vi "ReversedEngineering CreateEdges.vi"(1 "NodeRef":refnum<class "AbstractNode.lvclass">, 2 "AllNodes":refnum<class "AbstractNode.lvclass">[](array[class]), 3 "NodeClassInfo":T1, 5 "error in (no error)":errorcluster, 6 "Show Multiplicity":bool=TRUE) -> (15 "EdgesCreated":refnum<class "AbstractEdge.lvclass">[](array[class]), 19 "error out":errorcluster)   [LabVIEW 2020]
uses:
  <resource>/Framework/Providers/Open_GDS/UML/AbstractEdge_class/AbstractEdge.lvclass
  <resource>/Framework/Providers/Open_GDS/UML/AbstractNode_class/AbstractNode.lvclass
  <resource>/Framework/Providers/Open_GDS/UML/ReversedEngineering/ReversedEngineering ClassInfoType.ctl
  <resource>/Framework/Providers/Open_GDS/ClassProviders/Common/CommonVIs/CommonVIs_VisibilityType.ctl
  <resource>/Framework/Providers/Open_GDS/ClassProviders/Common/CommonVIs/CommonVIs_AttributeInfoType.ctl
  <resource>/Framework/Providers/Open_GDS/ClassProviders/Common/CommonVIs/CommonVIs_AttributeDataType.ctl
  <resource>/Framework/Providers/Open_GDS/UML/ReversedEngineering/ReversedEngineering_ClassDependencyDetailsType.ctl
  <resource>/Framework/Providers/Open_GDS/ClassProviders/Common/ScriptingFunctions/SubVIs/Scripting_ViDependencyType.ctl
  <resource>/Framework/Providers/Open_GDS/UML/ClassRelationshipEdge_class/ClassRelationshipEdge.lvclass
  C:/Program Files (x86)/National Instruments/LabVIEW 2020/resource/Framework/Providers/Open_GDS/UML/AbstractEdge_class/AbstractEdge.lvclass
  <resource>/Framework/Providers/Open_GDS/UML/ClassRelationshipEdge_class/ExternaSetParamType.ctl
  <resource>/Framework/Providers/Open_GDS/UML/ArrowHead_class/ArrowHeadType.ctl
  <resource>/Framework/Providers/Open_GDS/UML/BentStyle_class/BentStyleType.ctl
  <resource>/Framework/Providers/Open_GDS/UML/LineStyle_class/LineStyleType.ctl
  <resource>/Framework/Providers/Open_GDS/UML/ReversedEngineering/ReversedEngineering_ViDependencyDetailsType.ctl
  <resource>/Framework/Providers/Open_GDS/UML/ArrowHead_class/ArrowHead.lvclass
  <resource>/Framework/Providers/Open_GDS/UML/BentStyle_class/BentStyle.lvclass
  <resource>/Framework/Providers/Open_GDS/UML/LineStyle_class/LineStyle.lvclass
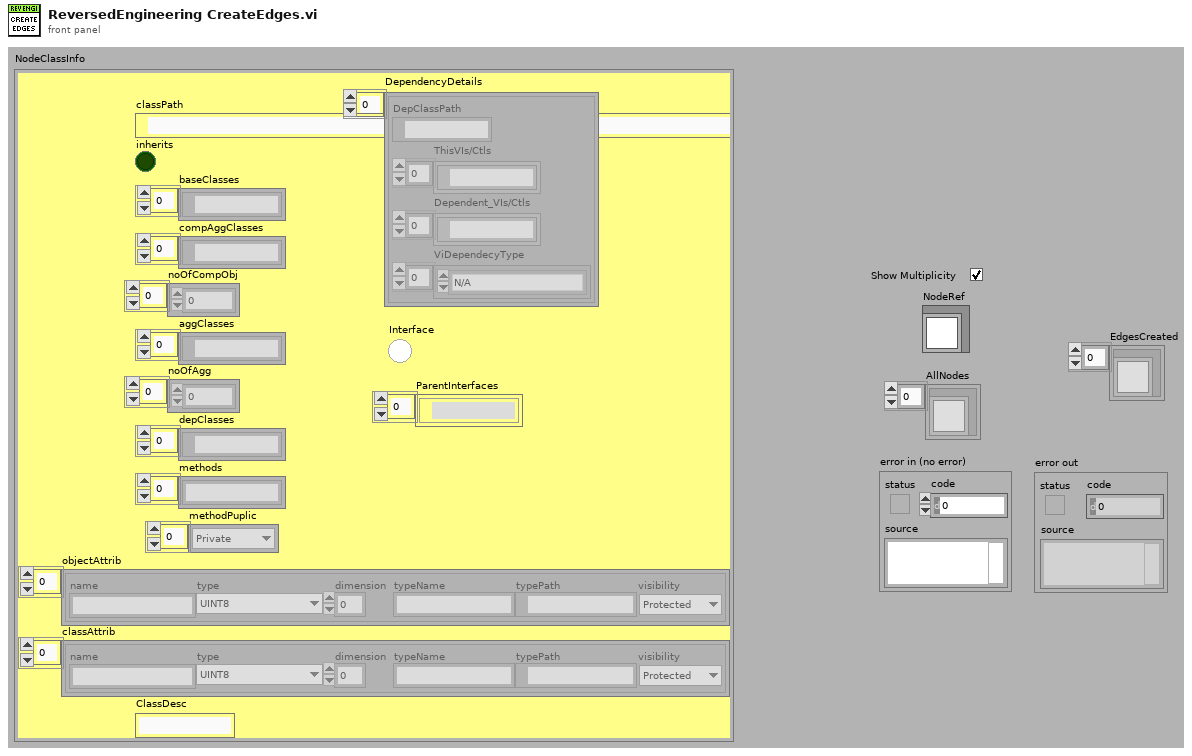
[diagram p1: front panel]
types:
  T1 = typedef "ReversedEngineering ClassInfoType.ctl" = cluster{"classPath":path, "inherits":bool, "baseClasses":path[], "compAggClasses":path[], "noOfCompObj":i32[], "aggClasses":path[], "noOfAgg":i32[], "depClasses":path[], "methods":string[], "methodPuplic":T2[], "objectAttrib":T3[], "classAttrib":T3[], "ClassDesc":string, "DependencyDetails":T5[], "Interface":bool, "ParentInterfaces":path[]}
  T2 = typedef "CommonVIs_VisibilityType.ctl" = enum16{"Public", "Private", "Protected"}
  T3 = typedef "CommonVIs_AttributeInfoType.ctl" = cluster{"name":string, "type":T4, "dimension":i32, "typeName":string, "typePath":path, "visibility":T2}
  T4 = typedef "CommonVIs_AttributeDataType.ctl" = enum16{"UINT8", "INT8", "UINT16", "INT16", "UINT32", "INT32", "UINT64", "INT64", "SGL", "DBL", "EXT", "CSG", "CDB", "CXT", "TimeStamp", "STRING", "PATH", "BOOL", "ENUM", "RefNum", "VIRefNum", "LabVIEW Class", "Cluster", "Variant", "TypeDef", "Waveform", "LabVIEW Object", "Other", "void", "Set", "Map"}
  T5 = typedef "ReversedEngineering_ClassDependencyDetailsType.ctl" = cluster{"DepClassPath":path, "ThisVIs/Ctls":path[], "Dependent_VIs/Ctls":path[], "ViDependecyType":T6[]}
  T6 = typedef "Scripting_ViDependencyType.ctl" = enum16{"N/A", "Launches"}
  T7 = typedef "ReversedEngineering_ViDependencyDetailsType.ctl" = cluster{"ThisVIs/Ctls":path[], "Dependent_VIs/Ctls":path[]}
  T8 = typedef "BentStyle.lvclass/BentStyleType.ctl" = enum16{"STRAIGHT", "HV", "VH", "HVH", "VHV", "ARC"}
  T9 = typedef "ClassRelationshipEdge.lvclass/ExternaSetParamType.ctl" = enum16{"StartLabel", "MidLabel", "EndLabel", "StartNode", "EndNode", "BendType", "StartArrow", "EndArrow", "StartOffset", "EndOffset", "LineStyle"}
  T10 = typedef "ArrowHead.lvclass/ArrowHeadType.ctl" = enum16{"NONE", "TRIANGLE", "BLACK_TRIANGLE", "V", "HALF_V", "DIAMOND", "BLACK_DIAMOND"}
  T11 = typedef "LineStyle.lvclass/LineStyleType.ctl" = enum16{"SOLID", "DOTTED"}
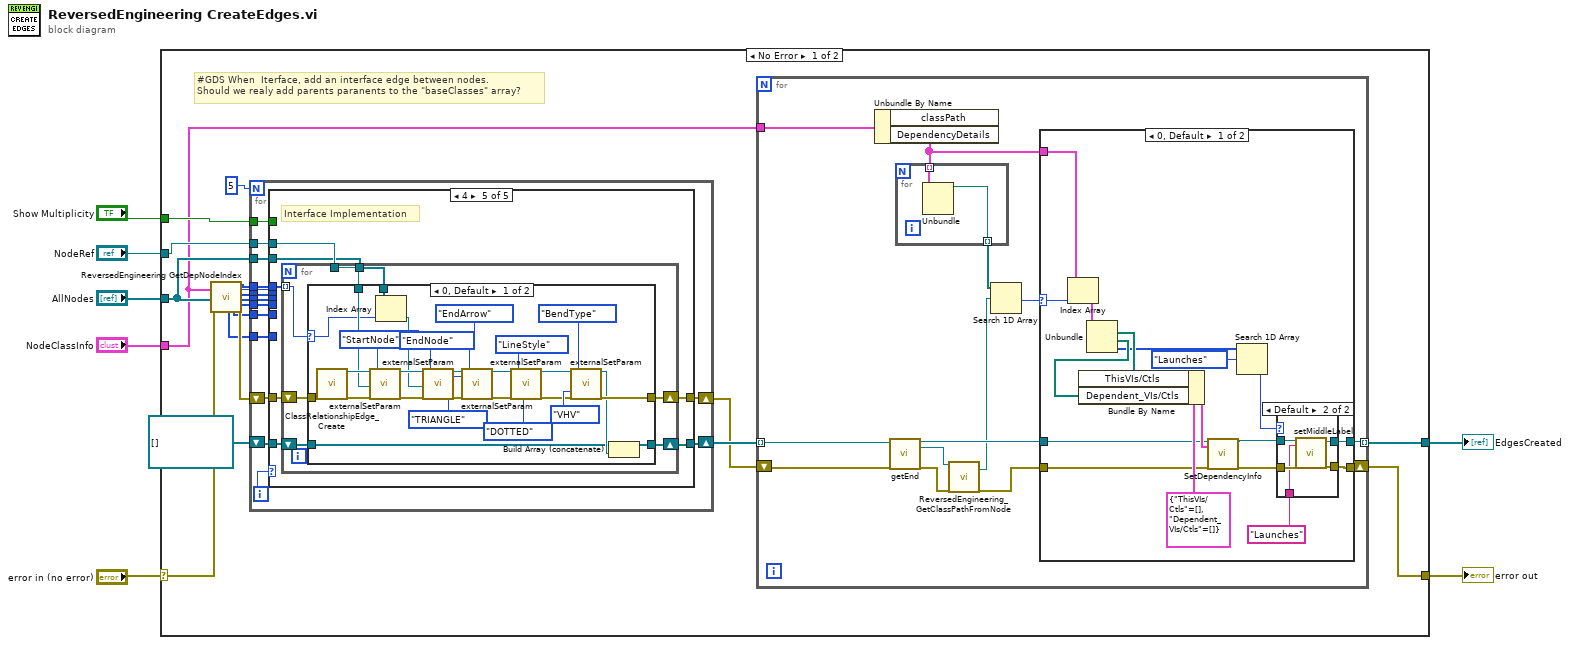
[diagram p0: block diagram]
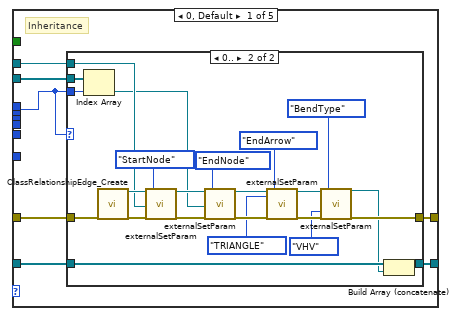
[diagram p4: hidden frame]
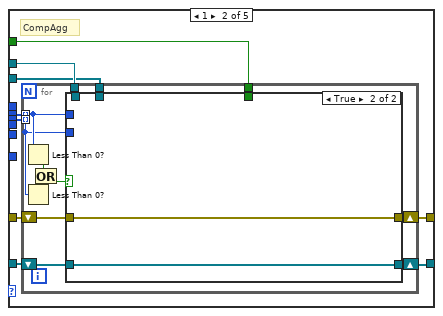
[diagram p6: hidden frame]
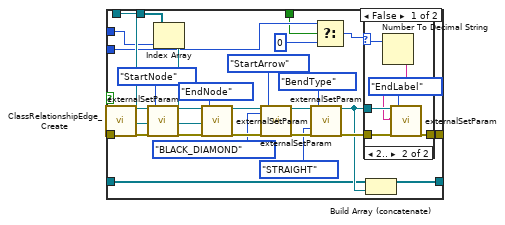
[diagram p7: hidden frame]
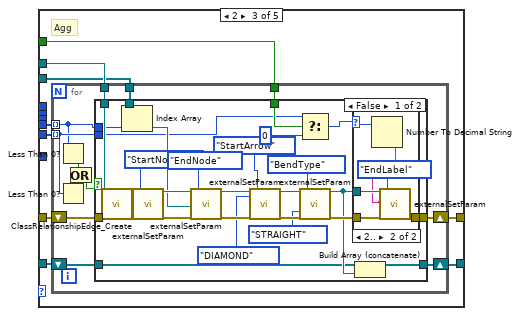
[diagram p9: hidden frame]
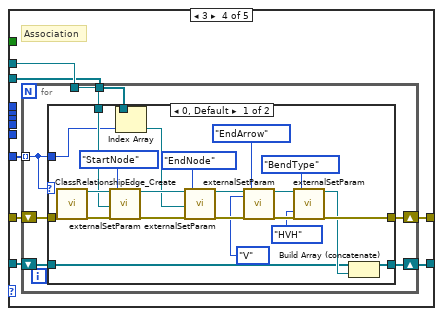
[diagram p12: hidden frame]
diagram:
  n1 = case shown="No Error" "error in (no error)" {
    selector: "error in (no error)" -> [w17 w313]
    tunnel: [w9 w313] -> w6
    tunnel: [w12 _] -> w5
    tunnel: "Show Multiplicity" -> [w16 _]
    tunnel: "AllNodes" -> [w14 _]
    tunnel: "NodeRef" -> [w15 _]
    tunnel: "NodeClassInfo" -> [w11 _]
    frame No Error {
      # "#GDS When  Iterface, add an interface edge between nodes.\nShould we realy add parents paranents to the \"baseClasses\" array?"
      n2 = call <resource>:"ReversedEngineering GetDepNodeIndex.vi"("classInfo"=w11, "AllNodes"=w14, "error in (no error)"=w17) -> ("depNodes"=w19:i32[], "noOfAgg"=w20:i32[], "InterfaceNodes"=w8:i32[], "inheritanceNode"=w24:i32, "compAggNodes"=w23:i32[], "noOfCompAgg"=w22:i32[], "aggNodes"=w21:i32[], "error out"=w25:errorcluster)  [unwired: 1 in, 8 out]
      n3 = for {
        N: 5 -> [_]
        tunnel: w15 -> [w82]
        shift-right: [w80] -> w10
        shift-left: w25 -> [w81]
        tunnel: w14 -> [w78]
        tunnel: w24 -> [w77]
        shift-right: [w76] -> w13
        shift-left: refnum<class "ClassRelationshipEdge.lvclass">[] [] ("empty") -> [w75]
        tunnel: w23 -> [w74]
        tunnel: w22 -> [w73]
        tunnel: w21 -> [w72]
        tunnel: w20 -> [w71]
        tunnel: w19 -> [w70]
        tunnel: w16 -> [w69]
        tunnel: w8 -> [w68]
        i -> [w79]
        n4 = case shown="4" w79 {
          tunnel: w81 -> [w89 w123 w181 w237 w276]
          tunnel: w82 -> [w88 w122 w180 w236 w275]
          tunnel: [w84 w121 w179 w235 w274] -> w80
          tunnel: w78 -> [w87 w119 w178 w234 w273]
          tunnel: w77 -> [w83 _ _ _ _]
          tunnel: [w86 w116 w176 w232 w271] -> w76
          tunnel: w75 -> [w85 w117 w177 w233 w272]
          tunnel: w74 -> [_ w120 _ _ _]
          tunnel: w73 -> [_ w118 _ _ _]
          tunnel: w72 -> [_ _ w175 _ _]
          tunnel: w71 -> [_ _ w174 _ _]
          tunnel: w70 -> [_ _ _ w231 _]
          tunnel: w69 -> [_ w115 w173 _ _]
          tunnel: w68 -> [_ _ _ _ w270]
          frame 0, Default {
            # "Inheritance"
            n5 = case shown="0.." w83 {
              tunnel: w89 -> [w91 w114]
              tunnel: w88 -> [_ w105]
              tunnel: w87 -> [_ w104]
              tunnel: w83 -> [_ w103]
              tunnel: [w90 w99] -> w86
              tunnel: w85 -> [w90 w98]
              tunnel: [w91 w95] -> w84
              frame Default {
              }
              frame 0.. {
                n6 = Index Array(array=w104, index=w103) -> (element=w102:refnum<class "AbstractNode.lvclass">)
                n7 = call <resource>:"ClassRelationshipEdge_Create.vi"("error in (no error)"=w114) -> ("reference out"=w113:refnum<class "ClassRelationshipEdge.lvclass">, "error out"=w112:errorcluster)  [unwired: 1 in, 16 out]
                n8 = call-dynamic "externalSetParam.vi"("reference"=w113, "node"=w105, "error in (no error)"=w112, "setParam"=ExternaSetParamType."StartNode") -> ("reference out"=w110:refnum<class "ClassRelationshipEdge.lvclass">, "error out"=w109:errorcluster)  [unwired: 14 in]
                n9 = call-dynamic "externalSetParam.vi"("reference"=w110, "node"=w102, "error in (no error)"=w109, "setParam"=ExternaSetParamType."EndNode") -> ("reference out"=w108:refnum<class "ClassRelationshipEdge.lvclass">, "error out"=w107:errorcluster)  [unwired: 14 in]
                n10 = call-dynamic "externalSetParam.vi"("reference"=w108, "arrowHead"=ArrowHeadType."TRIANGLE", "error in (no error)"=w107, "setParam"=ExternaSetParamType."EndArrow") -> ("reference out"=w97:refnum<class "ClassRelationshipEdge.lvclass">, "error out"=w96:errorcluster)  [unwired: 14 in]
                n11 = call-dynamic "externalSetParam.vi"("reference"=w97, "bentStyle"=BentStyleType."VHV", "error in (no error)"=w96, "setParam"=ExternaSetParamType."BendType") -> ("reference out"=w94:refnum<class "ClassRelationshipEdge.lvclass">, "error out"=w95:errorcluster)  [unwired: 14 in]
                n12 = Build Array (concatenate)(w98, w94) -> (w99:refnum<class "ClassRelationshipEdge.lvclass">[])
              }
            }
          }
          frame 1 {
            # "CompAgg"
            n13 = for {
              shift-right: [w133] -> w121
              shift-left: w123 -> [w135]
              tunnel: w122 -> [w134]
              tunnel: w120 -> [w128] mode=indexing
              tunnel: w119 -> [w132]
              tunnel: w118 -> [w127] mode=indexing
              shift-right: [w130] -> w116
              shift-left: w117 -> [w131]
              tunnel: w115 -> [w129]
              n14 = Less Than 0?(x=w128) -> (x < 0?=w126:bool)
              n15 = Less Than 0?(x=w127) -> (x < 0?=w125:bool)
              n16 = Or(x=w126, y=w125) -> (x .or. y?=w124:bool)
              n17 = case shown="True" w124 {
                tunnel: w135 -> [w152 w172]
                tunnel: w134 -> [w151 _]
                tunnel: [w150 w172] -> w133
                tunnel: w128 -> [w149 _]
                tunnel: w132 -> [w148 _]
                tunnel: w131 -> [w142 w171]
                tunnel: [w141 w171] -> w130
                tunnel: w127 -> [w138 _]
                tunnel: w129 -> [w137 _]
                frame False {
                  n18 = call <resource>:"ClassRelationshipEdge_Create.vi"("error in (no error)"=w152) -> ("reference out"=w163:refnum<class "ClassRelationshipEdge.lvclass">, "error out"=w162:errorcluster)  [unwired: 1 in, 16 out]
                  n19 = call-dynamic "externalSetParam.vi"("reference"=w163, "node"=w151, "error in (no error)"=w162, "setParam"=ExternaSetParamType."StartNode") -> ("reference out"=w160:refnum<class "ClassRelationshipEdge.lvclass">, "error out"=w159:errorcluster)  [unwired: 14 in]
                  n20 = Index Array(array=w148, index=w149) -> (element=w147:refnum<class "AbstractNode.lvclass">)
                  n21 = call-dynamic "externalSetParam.vi"("reference"=w160, "node"=w147, "error in (no error)"=w159, "setParam"=ExternaSetParamType."EndNode") -> ("reference out"=w158:refnum<class "ClassRelationshipEdge.lvclass">, "error out"=w157:errorcluster)  [unwired: 14 in]
                  n22 = call-dynamic "externalSetParam.vi"("reference"=w158, "arrowHead"=ArrowHeadType."BLACK_DIAMOND", "error in (no error)"=w157, "setParam"=ExternaSetParamType."StartArrow") -> ("reference out"=w156:refnum<class "ClassRelationshipEdge.lvclass">, "error out"=w155:errorcluster)  [unwired: 14 in]
                  n23 = call-dynamic "externalSetParam.vi"("reference"=w156, "bentStyle"=BentStyleType."STRAIGHT", "error in (no error)"=w155, "setParam"=ExternaSetParamType."BendType") -> ("reference out"=w143:refnum<class "ClassRelationshipEdge.lvclass">, "error out"=w154:errorcluster)  [unwired: 14 in]
                  n24 = Select(t=w138, s=w137, f=0) -> (s? t:f=w139:i32)
                  n25 = case shown="2.." w139 {
                    selector: w139 -> [_ w167]
                    tunnel: w143 -> [_ w170]
                    tunnel: w154 -> [w164 w169]
                    tunnel: [w164 w168] -> w150
                    frame 0, Default {
                    }
                    frame 2.. {
                      n26 = Number To Decimal String(number=w167) -> (decimal integer string=w166:string)  [unwired: 1 out]
                      n27 = call-dynamic "externalSetParam.vi"("reference"=w170, "string"=w166, "error in (no error)"=w169, "setParam"=ExternaSetParamType."EndLabel") -> ("error out"=w168:errorcluster)  [unwired: 14 in, 1 out]
                    }
                  }
                  n28 = Build Array (concatenate)(w142, w143) -> (w141:refnum<class "ClassRelationshipEdge.lvclass">[])
                }
                frame True {
                }
              }
            }
          }
          frame 2 {
            # "Agg"
            n29 = for {
              shift-right: [w191] -> w179
              shift-left: w181 -> [w193]
              tunnel: w180 -> [w192]
              tunnel: w175 -> [w183] mode=indexing
              tunnel: w178 -> [w190]
              tunnel: w174 -> [w184] mode=indexing
              shift-right: [w188] -> w176
              shift-left: w177 -> [w189]
              tunnel: w173 -> [w187]
              n30 = Less Than 0?(x=w183) -> (x < 0?=w186:bool)
              n31 = Less Than 0?(x=w184) -> (x < 0?=w185:bool)
              n32 = Or(x=w186, y=w185) -> (x .or. y?=w182:bool)
              n33 = case shown="False" w182 {
                tunnel: w193 -> [w210 w230]
                tunnel: w192 -> [w209 _]
                tunnel: [w208 w230] -> w191
                tunnel: w190 -> [w207 _]
                tunnel: w189 -> [w200 w229]
                tunnel: [w199 w229] -> w188
                tunnel: w187 -> [w196 _]
                tunnel: w184 -> [w195 _]
                tunnel: w183 -> [w194 _]
                frame False {
                  n34 = call <resource>:"ClassRelationshipEdge_Create.vi"("error in (no error)"=w210) -> ("reference out"=w221:refnum<class "ClassRelationshipEdge.lvclass">, "error out"=w220:errorcluster)  [unwired: 1 in, 16 out]
                  n35 = Index Array(array=w207, index=w194) -> (element=w206:refnum<class "AbstractNode.lvclass">)
                  n36 = call-dynamic "externalSetParam.vi"("reference"=w221, "node"=w209, "error in (no error)"=w220, "setParam"=ExternaSetParamType."StartNode") -> ("reference out"=w218:refnum<class "ClassRelationshipEdge.lvclass">, "error out"=w217:errorcluster)  [unwired: 14 in]
                  n37 = call-dynamic "externalSetParam.vi"("reference"=w218, "node"=w206, "error in (no error)"=w217, "setParam"=ExternaSetParamType."EndNode") -> ("reference out"=w216:refnum<class "ClassRelationshipEdge.lvclass">, "error out"=w215:errorcluster)  [unwired: 14 in]
                  n38 = call-dynamic "externalSetParam.vi"("reference"=w216, "arrowHead"=ArrowHeadType."DIAMOND", "error in (no error)"=w215, "setParam"=ExternaSetParamType."StartArrow") -> ("reference out"=w214:refnum<class "ClassRelationshipEdge.lvclass">, "error out"=w213:errorcluster)  [unwired: 14 in]
                  n39 = Select(t=w195, s=w196, f=0) -> (s? t:f=w197:i32)
                  n40 = call-dynamic "externalSetParam.vi"("reference"=w214, "bentStyle"=BentStyleType."STRAIGHT", "error in (no error)"=w213, "setParam"=ExternaSetParamType."BendType") -> ("reference out"=w201:refnum<class "ClassRelationshipEdge.lvclass">, "error out"=w212:errorcluster)  [unwired: 14 in]
                  n41 = case shown="2.." w197 {
                    selector: w197 -> [_ w225]
                    tunnel: w201 -> [_ w228]
                    tunnel: w212 -> [w222 w227]
                    tunnel: [w222 w226] -> w208
                    frame 0, Default {
                    }
                    frame 2.. {
                      n42 = Number To Decimal String(number=w225) -> (decimal integer string=w224:string)  [unwired: 1 out]
                      n43 = call-dynamic "externalSetParam.vi"("reference"=w228, "string"=w224, "error in (no error)"=w227, "setParam"=ExternaSetParamType."EndLabel") -> ("error out"=w226:errorcluster)  [unwired: 14 in, 1 out]
                    }
                  }
                  n44 = Build Array (concatenate)(w200, w201) -> (w199:refnum<class "ClassRelationshipEdge.lvclass">[])
                }
                frame True {
                }
              }
            }
          }
          frame 3 {
            # "Association"
            n45 = for {
              shift-right: [w242] -> w235
              shift-left: w237 -> [w244]
              tunnel: w236 -> [w243]
              tunnel: w234 -> [w241]
              shift-right: [w239] -> w232
              shift-left: w233 -> [w240]
              tunnel: w231 -> [w238] mode=indexing
              n46 = case shown="0, Default" w238 {
                tunnel: w244 -> [w257 w269]
                tunnel: w243 -> [w256 _]
                tunnel: [w255 w269] -> w242
                tunnel: w241 -> [w254 _]
                tunnel: w240 -> [w247 w268]
                tunnel: [w246 w268] -> w239
                tunnel: w238 -> [w245 _]
                frame 0, Default {
                  n47 = call <resource>:"ClassRelationshipEdge_Create.vi"("error in (no error)"=w257) -> ("reference out"=w267:refnum<class "ClassRelationshipEdge.lvclass">, "error out"=w266:errorcluster)  [unwired: 1 in, 16 out]
                  n48 = call-dynamic "externalSetParam.vi"("reference"=w267, "node"=w256, "error in (no error)"=w266, "setParam"=ExternaSetParamType."StartNode") -> ("reference out"=w264:refnum<class "ClassRelationshipEdge.lvclass">, "error out"=w263:errorcluster)  [unwired: 14 in]
                  n49 = Index Array(array=w254, index=w245) -> (element=w253:refnum<class "AbstractNode.lvclass">)
                  n50 = call-dynamic "externalSetParam.vi"("reference"=w264, "node"=w253, "error in (no error)"=w263, "setParam"=ExternaSetParamType."EndNode") -> ("reference out"=w262:refnum<class "ClassRelationshipEdge.lvclass">, "error out"=w261:errorcluster)  [unwired: 14 in]
                  n51 = call-dynamic "externalSetParam.vi"("reference"=w262, "arrowHead"=ArrowHeadType."V", "error in (no error)"=w261, "setParam"=ExternaSetParamType."EndArrow") -> ("reference out"=w260:refnum<class "ClassRelationshipEdge.lvclass">, "error out"=w259:errorcluster)  [unwired: 14 in]
                  n52 = call-dynamic "externalSetParam.vi"("reference"=w260, "bentStyle"=BentStyleType."HVH", "error in (no error)"=w259, "setParam"=ExternaSetParamType."BendType") -> ("reference out"=w248:refnum<class "ClassRelationshipEdge.lvclass">, "error out"=w255:errorcluster)  [unwired: 14 in]
                  n53 = Build Array (concatenate)(w247, w248) -> (w246:refnum<class "ClassRelationshipEdge.lvclass">[])
                }
                frame -1 {
                }
              }
            }
          }
          frame 4 {
            # "Interface Implementation"
            n54 = for {
              shift-right: [w281] -> w274
              shift-left: w276 -> [w283]
              tunnel: w275 -> [w282]
              tunnel: w273 -> [w280]
              shift-right: [w278] -> w271
              shift-left: w272 -> [w279]
              tunnel: w270 -> [w277] mode=indexing
              n55 = case shown="0, Default" w277 {
                selector: w277 -> [w290 _]
                tunnel: w283 -> [w302 w312]
                tunnel: w282 -> [w301 _]
                tunnel: [w300 w312] -> w281
                tunnel: w280 -> [w299 _]
                tunnel: w279 -> [w292 w311]
                tunnel: [w291 w311] -> w278
                frame 0, Default {
                  n56 = call <resource>:"ClassRelationshipEdge_Create.vi"("error in (no error)"=w302) -> ("reference out"=w310:refnum<class "ClassRelationshipEdge.lvclass">, "error out"=w309:errorcluster)  [unwired: 1 in, 16 out]
                  n57 = call-dynamic "externalSetParam.vi"("reference"=w310, "node"=w301, "error in (no error)"=w309, "setParam"=ExternaSetParamType."StartNode") -> ("reference out"=w307:refnum<class "ClassRelationshipEdge.lvclass">, "error out"=w306:errorcluster)  [unwired: 14 in]
                  n58 = Index Array(array=w299, index=w290) -> (element=w298:refnum<class "AbstractNode.lvclass">)
                  n59 = call-dynamic "externalSetParam.vi"("reference"=w307, "node"=w298, "error in (no error)"=w306, "setParam"=ExternaSetParamType."EndNode") -> ("reference out"=w305:refnum<class "ClassRelationshipEdge.lvclass">, "error out"=w304:errorcluster)  [unwired: 14 in]
                  n60 = call-dynamic "externalSetParam.vi"("reference"=w305, "arrowHead"=ArrowHeadType."TRIANGLE", "error in (no error)"=w304, "setParam"=ExternaSetParamType."EndArrow") -> ("reference out"=w289:refnum<class "ClassRelationshipEdge.lvclass">, "error out"=w288:errorcluster)  [unwired: 14 in]
                  n61 = call-dynamic "externalSetParam.vi"("reference"=w289, "error in (no error)"=w288, "setParam"=ExternaSetParamType."LineStyle", "lineStyle"=LineStyleType."DOTTED") -> ("reference out"=w286:refnum<class "ClassRelationshipEdge.lvclass">, "error out"=w287:errorcluster)  [unwired: 14 in]
                  n62 = call-dynamic "externalSetParam.vi"("reference"=w286, "bentStyle"=BentStyleType."VHV", "error in (no error)"=w287, "setParam"=ExternaSetParamType."BendType") -> ("reference out"=w293:refnum<class "ClassRelationshipEdge.lvclass">, "error out"=w300:errorcluster)  [unwired: 14 in]
                  n63 = Build Array (concatenate)(w292, w293) -> (w291:refnum<class "ClassRelationshipEdge.lvclass">[])
                }
                frame -1 {
                }
              }
            }
          }
        }
      }
      n64 = for {
        tunnel: w13 -> [w27] mode=indexing
        tunnel: [w38] -> w12 mode=indexing
        tunnel: w11 -> [w39]
        shift-right: [w37] -> w9
        shift-left: w10 -> [w28]
        n65 = Unbundle By Name(w39) -> ("DependencyDetails"=w29:T5[])  [unwired: 1 out]
        n66 = call-dynamic "getEnd.vi"("reference"=w27, "error in (no error)"=w28) -> ("reference out"=w34:refnum<class "ClassRelationshipEdge.lvclass">, "endNode"=w35:refnum<class "AbstractNode.lvclass">, "error out"=w36:errorcluster)  [unwired: 14 in, 1 out]
        n67 = for {
          tunnel: w29 -> [w67] mode=indexing
          tunnel: [w66] -> w33 mode=indexing
          n68 = Unbundle(w67) -> ("DepClassPath"=w66:path)  [unwired: 3 out]
        }
        n69 = call <resource>:"ReversedEngineering_GetClassPathFromNode.vi"("reference"=w35, "error IO"=w36) -> ("Path"=w32:path, "error out"=w30:errorcluster)  [unwired: 2 in, 14 out]
        n70 = Search 1D Array(1D array=w33, element=w32) -> (index of element=w31:i32)  [unwired: 1 out]
        n71 = case shown="0, Default" w31 {
          selector: w31 -> [w52 _]
          tunnel: [w42 w65] -> w38
          tunnel: [w43 w64] -> w37
          tunnel: w34 -> [w54 w65]
          tunnel: w30 -> [w53 w64]
          tunnel: w29 -> [w51 _]
          frame 0, Default {
            n72 = Index Array(array=w51, index=w52) -> (element=w50:T5)
            n73 = Unbundle(w50) -> ("ThisVIs/Ctls"=w49:path[], "Dependent_VIs/Ctls"=w48:path[], "ViDependecyType"=w47:T6[])  [unwired: 1 out]
            n74 = Bundle By Name(cluster=T7 {"ThisVIs/Ctls"=[], "Dependent_VIs/Ctls"=[]} ("DepClass"), "ThisVIs/Ctls"=w49, "Dependent_VIs/Ctls"=w48) -> (w55:T7)
            n75 = call <resource>:"SetDependencyInfo.vi"("reference"=w54, "DepClass"=w55, "error in (no error)"=w53) -> ("reference out"=w45:refnum<class "ClassRelationshipEdge.lvclass">, "error out"=w44:errorcluster)  [unwired: 15 out]
            n76 = Search 1D Array(1D array=w47, element=Scripting_ViDependencyType."Launches") -> (index of element=w41:i32)  [unwired: 1 in]
            n77 = case shown="Default" w41 {
              tunnel: w45 -> [w58 w63]
              tunnel: w44 -> [w57 w62]
              tunnel: [w57 w61] -> w43
              tunnel: [w58 w60] -> w42
              tunnel: "Launches" ("middleLabel") -> [_ w59]
              frame -1 {
              }
              frame Default {
                n78 = call-dynamic "setMiddleLabel.vi"("reference"=w63, "middleLabel"=w59, "error in (no error)"=w62) -> ("reference out"=w60:refnum<class "ClassRelationshipEdge.lvclass">, "error out"=w61:errorcluster)  [unwired: 15 in]
              }
            }
          }
          frame -1 {
          }
        }
      }
    }
    frame Error {
    }
  }
  "error out" <- w6
  "EdgesCreated" <- w5
